vi "Connect.vi"(8 "error in (no error)":errorcluster, 10 "Connection String":string, 11 "dbcDotNet Type":refnum<class "ORM_DBC_dotNetCore.lvclass">) -> (0 "error out":errorcluster, 3 "dbcDotNet out":refnum<class "ORM_DBC_dotNetCore.lvclass">)   [LabVIEW 2026, in "ORM_DBC_dotNetCore.lvlib" / "ORM_DBC_dotNetCore.lvclass"]
uses:
  ORM_DBC_dotNetCore.lvclass
  <vilib>/Viviota/shared/ORM.lvlibp/DbConnection/DbConnection.lvclass
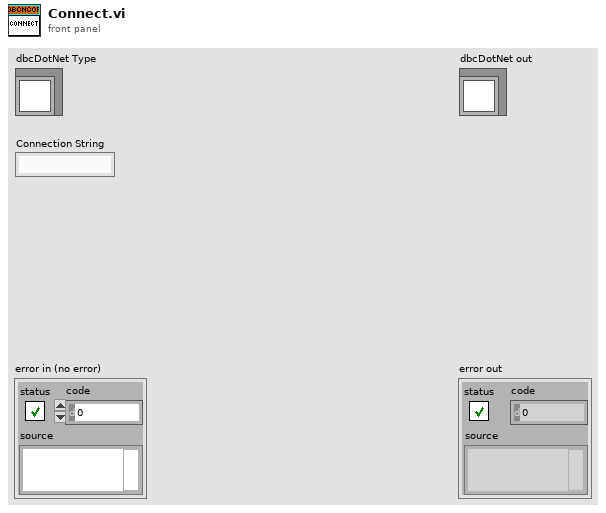
[diagram p1: front panel]
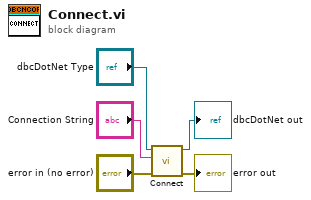
[diagram p0: block diagram]
diagram:
  n1 = call-parent "Connect.vi"("error in (no error)"="error in (no error)", "Connection String"="Connection String", "DbConnection Type"="dbcDotNet Type") -> ("error out"=→"error out":errorcluster, "DbConnection out"=→"dbcDotNet out":refnum<class "ORM_DBC_dotNetCore.lvclass">)  [unwired: 7 in]
